vi "Path Type Specialization - Multiple Converter.vi"(11 "error in":errorcluster) -> (4 "type specialization for path":T1(array[cluster]), 15 "error out":errorcluster)   [LabVIEW 2021, in "Converter.lvlib"]
uses:
  Converter.lvlib
  <vilib>/Utility/traverseref.llb/TRef TravTarget.ctl
  <vilib>/Utility/traverseref.llb/VI Scripting - Traverse.lvlib
  Path Functions/Path Functions.lvlib
  Converter Reusables/Converter Reusables.lvlib
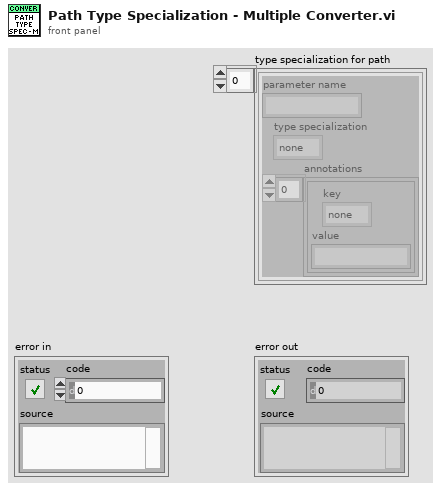
[diagram p1: front panel]
types:
  T1 = cluster{"parameter name":string, "type specialization":enum16{"none", "pin", "path", "enum"}, "annotations":cluster{"key":enum16{"none", "pin.instrument_type", "enum.values"}, "value":string}[]}[]
  T2 = typedef "TRef TravTarget.ctl" = enum16{"FP", "BD", "Other"}
  T3 = cluster{"parameter name":string, "type specialization":enum16{"none", "pin", "path", "enum"}, "annotations":cluster{"key":enum16{"none", "pin.instrument_type", "enum.values"}, "value":string}[]}
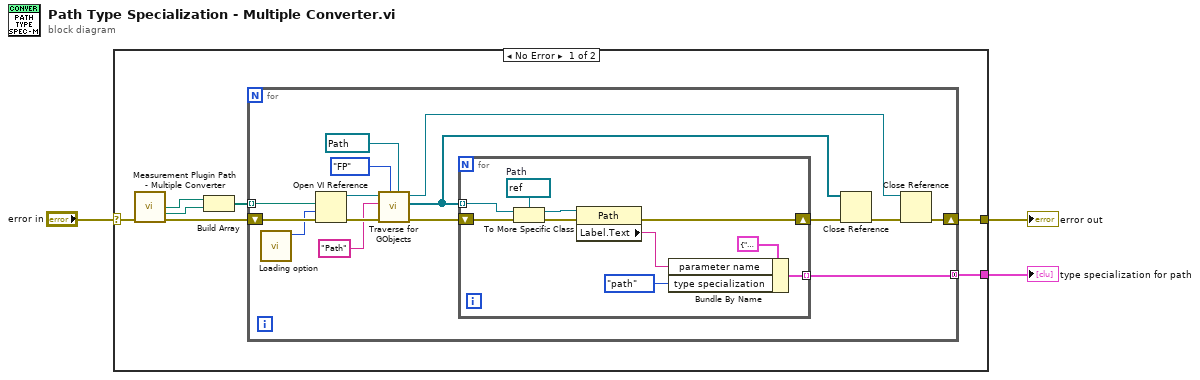
[diagram p0: block diagram]
diagram:
  n1 = case shown="No Error" "error in" {
    selector: "error in" -> [w10 w36]
    tunnel: [w5 w36] -> w2
    tunnel: [w4 _] -> w1
    frame No Error {
      n2 = call "Measurement Plugin Path - Multiple Converter.vi"("error in"=w10) -> ("result control"=w8:path, "input controls"=w7:path, "error out"=w9:errorcluster)  [unwired: 2 in, 10 out]
      n3 = Build Array(w8, w7) -> (w6:path[])
      n4 = for {
        tunnel: w6 -> [w13] mode=indexing
        shift-right: [w15] -> w5
        shift-left: w9 -> [w24]
        tunnel: [w19] -> w4 mode=concatenating
        n5 = call "Loading option.vi"() -> ("options"=w11:i32)  [unwired: 11 in]
        n6 = Open VI Reference(vi path=w13, options=w11, error in (no error)=w24) -> (vi reference=w23:refnum<vi>, error out=w25:errorcluster)  [unwired: 3 in]
        n7 = call <vilib>:"Traverse for GObjects.vi"("Other Refnum"=refnum<vi> refnum, "Traverse Target"=TRef_TravTarget."FP", "error in (no error)"=w25, "Class Name"="Path", "VI Refnum"=w23) -> ("error out"=w20:errorcluster, "References"=w17:refnum<vi>[], "dup VI Refnum"=w16:refnum<vi>)  [unwired: 3 in, 1 out]
        n8 = for {
          shift-right: [w29] -> w18
          shift-left: w20 -> [w35]
          tunnel: w17 -> [w34] mode=indexing
          tunnel: [w28] -> w19 mode=indexing
          w26 = refnum<vi> refnum  # Path
          n9 = To More Specific Class(target class=w26, reference=w34, error in=w35) -> (specific class reference=w32:refnum<vi>, error out=w33:errorcluster)
          n10 = property class="Path"(reference=w32, error in=w33) -> (error out=w29:errorcluster, "Label.Text"=w30:string)  [unwired: 1 out]
          n11 = Bundle By Name(cluster=T3 {"parameter name"="", "type specialization"=enum."none", "annotations"=[]} ("Type Specialization"), "parameter name"=w30, "type specialization"=enum16{"none", "pin", "path", "enum"}."path") -> (w28:T3)
        }
        n12 = Close Reference(reference=w17, error in (no error)=w18) -> (error out=w14:errorcluster)
        n13 = Close Reference(reference=w16, error in (no error)=w14) -> (error out=w15:errorcluster)
      }
    }
    frame Error {
    }
  }
  "error out" <- w2
  "type specialization for path" <- w1
